vi "SubscribeSetPointUpdated Send Stream.vi"(10 "Temperature Set Point":dbl, 11 "Stream Data in":T1={"gRPCid"=0, "Active"=FALSE, "timeout"=-1}) -> (0 "error out":errorcluster)   [LabVIEW 2020]
doc: "Send data with <b>Streaming?</b> parameter set to True to maintain stream active."
uses:
  Stream Data--cluster.ctl
  <vilib>/gRPC/LabVIEW gRPC Library/Shared/grpcId.ctl
  thermal-chamber-controller_server/RPC Messages/lv_python_grpc_webui_demo_v1_SetPointUpdated.ctl
  thermal-chamber-controller_server/thermal-chamber-controller_server.lvlib
  thermal-chamber-controller_server/RPC Service/ThermalChamberController/ThermalChamberController.lvclass
  <vilib>/gRPC/LabVIEW gRPC Library/grpc-lvsupport-release.lvlib
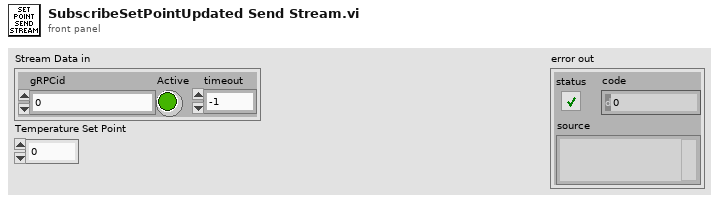
[diagram p1: front panel]
types:
  T1 = typedef "Stream Data--cluster.ctl" = cluster{"gRPCid":T2, "Active":bool, "timeout":i32}
  T2 = typedef "grpc-lvsupport-release.lvlib/grpcId.ctl" = u64
  T3 = typedef "thermal-chamber-controller_server.lvlib/lv_python_grpc_webui_demo_v1_SetPointUpdated.ctl" = cluster{"temperature_set_point":dbl}
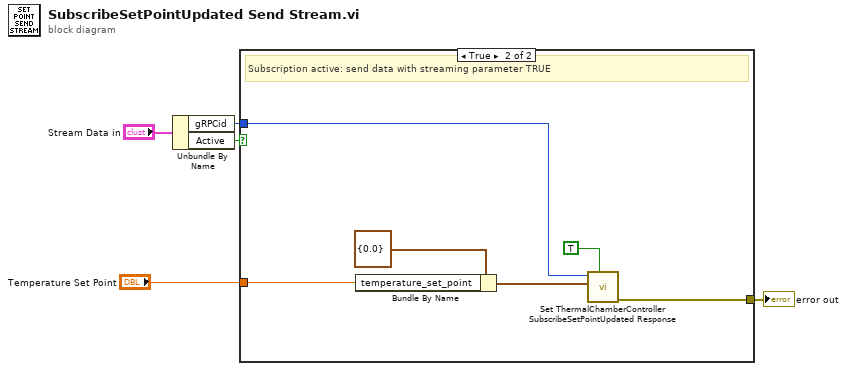
[diagram p0: block diagram]
diagram:
  n1 = Unbundle By Name("Stream Data in") -> ("gRPCid"=w4:T2, "Active"=w5:bool)
  n2 = case shown="True" w5 {
    tunnel: w4 -> [_ w11]
    tunnel: [_ w9] -> w1
    tunnel: "Temperature Set Point" -> [_ w7]
    frame False {
      # "Inactive: no action."
    }
    frame True {
      # "Subscription active: send data with streaming parameter TRUE"
      n3 = Bundle By Name(cluster=T3 {"temperature_set_point"=0.0} ("Message Data"), "temperature_set_point"=w7) -> (w6:T3)
      n4 = call "Set ThermalChamberController SubscribeSetPointUpdated Response.vi"("Streaming? (F)"=TRUE, "Message Data"=w6, "gRPCid in"=w11) -> ("error out"=w9:errorcluster)  [unwired: 8 in]
    }
  }
  "error out" <- w1
